vi "RelayControl.vi"(0 "Relay Task":refnum<k21>, 5 "error in":errorcluster, 7 "Battery Select (0: Off)":i32, 9 "NHR VISA":refnum<visa-resource-name>, 11 "NHR error in":errorcluster caption="NHR error in (no error)") -> (6 "error out":errorcluster, 10 "NHR Visa out":refnum<visa-resource-name>, 15 "NHR error out":errorcluster)   [LabVIEW 2020]
uses:
  <vilib>/DAQmx/write.llb/DAQmx Write (Digital 1D Bool NChan 1Samp 1Line).vi
  <vilib>/DAQmx/miscellaneous.llb/DAQmx Fill In Error Info.vi
  <instrlib>/NH Research Regenerative Test Series/NH Research Regenerative Test Series.lvlib
panel:
  out "String":string
  out "error out 3":errorcluster
  out "error out 2":errorcluster
  # "0:off, 1:B1 NHR, 2:B2 NHR, 3:B3 NHR, 4:3P NHR, 5:B1 BK, 6:B2 BK, 7:B3 BK, 8:3P BK"
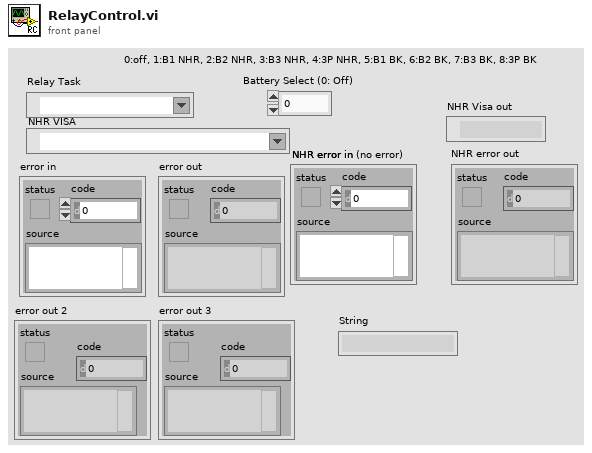
[diagram p1: front panel]
types:
  T1 = cluster{bool, bool, bool, bool, bool, bool, bool}
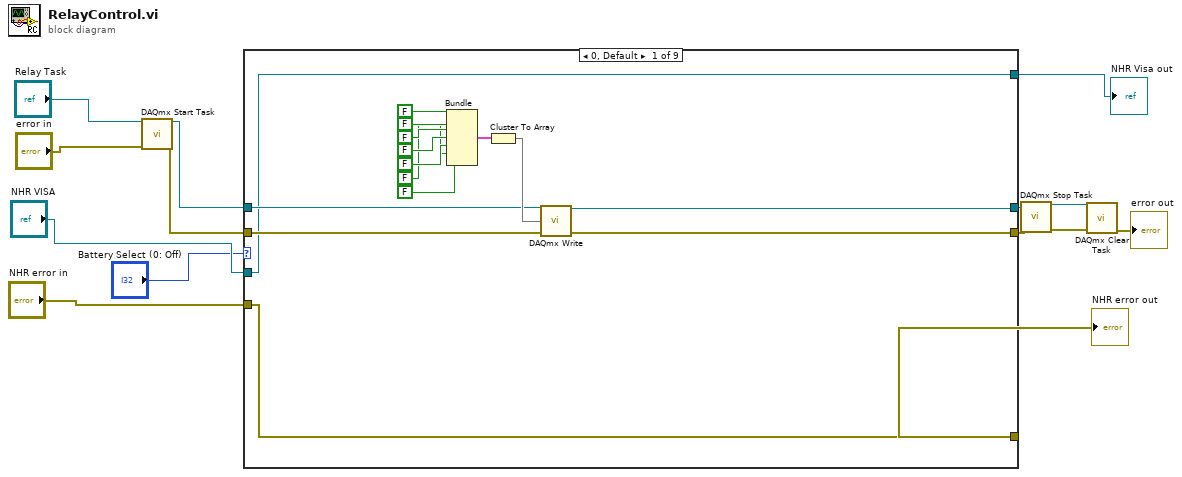
[diagram p0: block diagram]
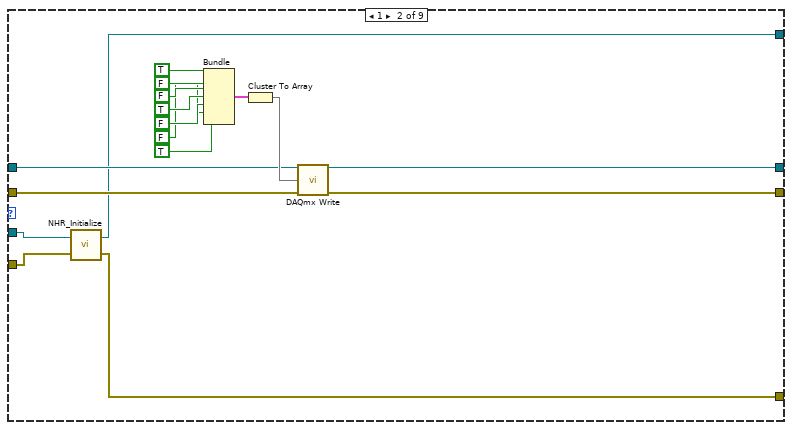
[diagram p2: hidden frame]
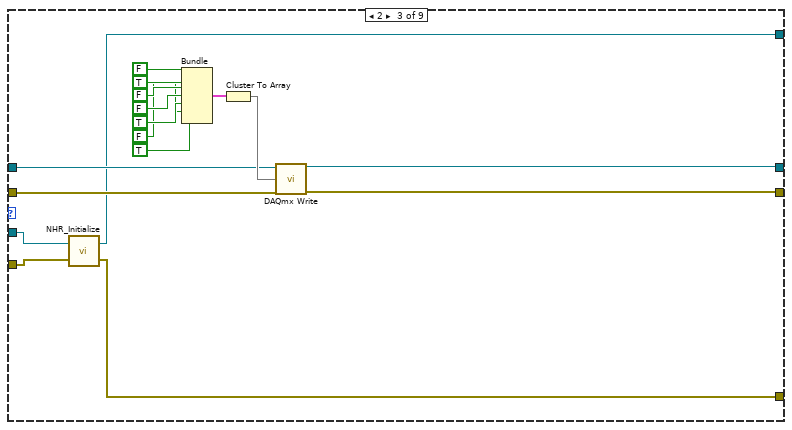
[diagram p3: hidden frame]
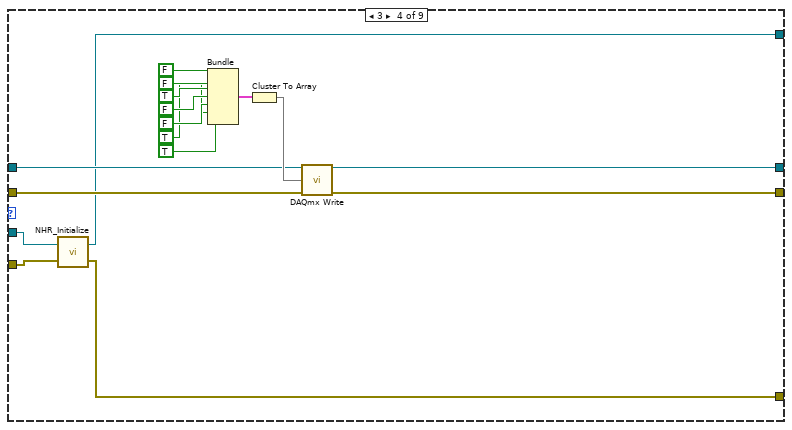
[diagram p4: hidden frame]
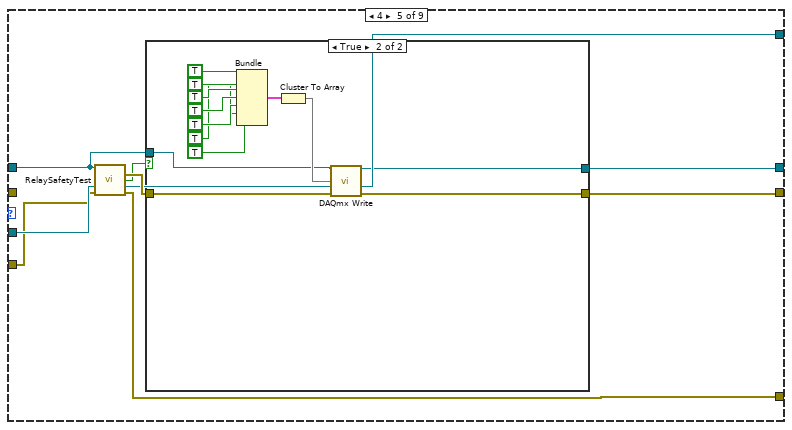
[diagram p5: hidden frame]
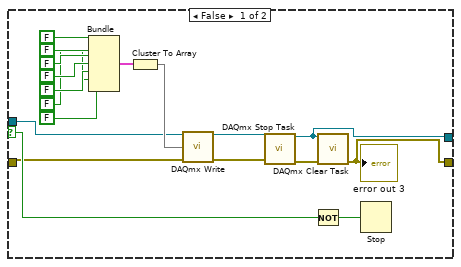
[diagram p6: hidden frame]
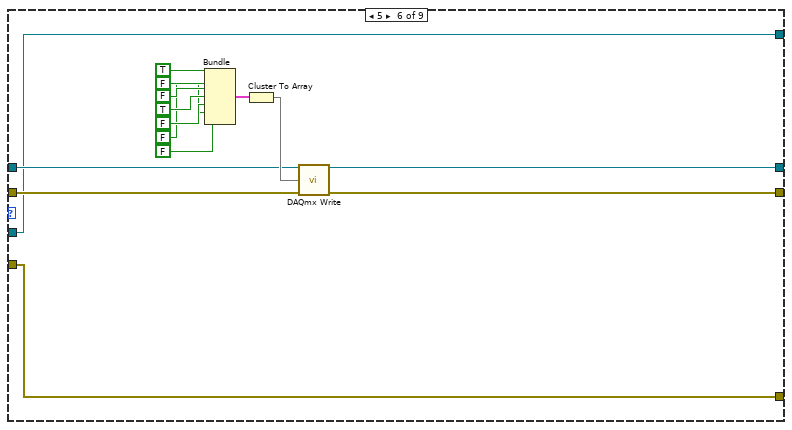
[diagram p7: hidden frame]
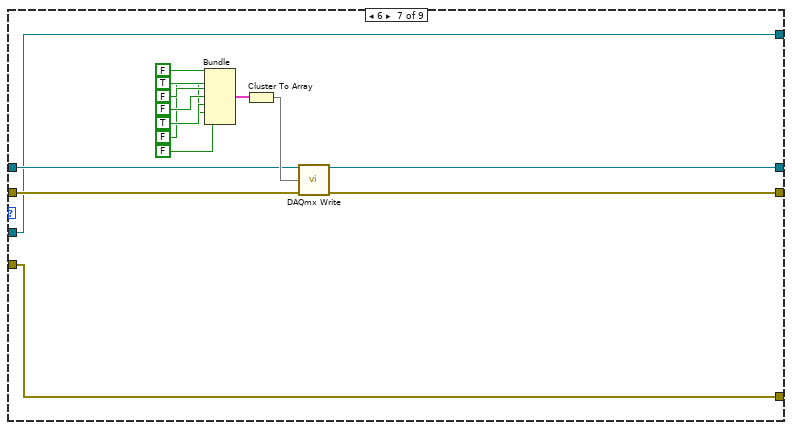
[diagram p8: hidden frame]
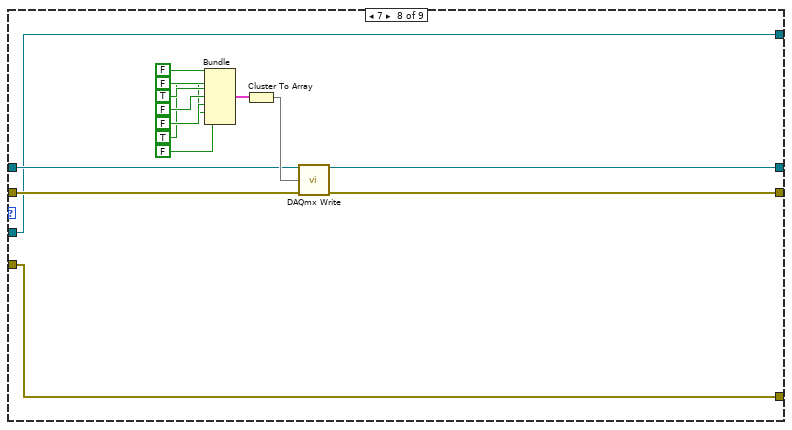
[diagram p9: hidden frame]
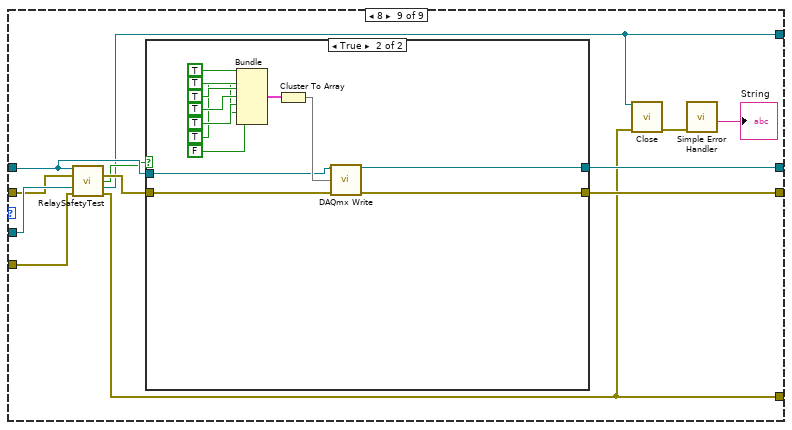
[diagram p10: hidden frame]
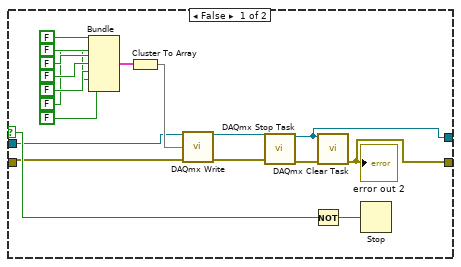
[diagram p11: hidden frame]
diagram:
  n1 = call <vilib>:"DAQmx Start Task.vi"("task/channels in"="Relay Task", "error in"="error in") -> ("task out"=w13:refnum<k21>, "error out"=w12:errorcluster)  [unwired: 12 in]
  n2 = case shown="0, Default" "Battery Select (0: Off)" {
    tunnel: w13 -> [w20 w37 w54 w71 w87 w126 w141 w156 w173]
    tunnel: w12 -> [w19 w36 w53 w70 _ w125 w140 w155 w174]
    tunnel: [w18 w35 w52 w69 w89 w124 w139 w154 w177] -> w8
    tunnel: [w17 w34 w51 w68 w88 w123 w138 w153 w167] -> w7
    tunnel: "NHR VISA" -> [w16 w33 w50 w67 w83 w122 w137 w152 w176]
    tunnel: "NHR error in" -> [w15 w32 w49 w66 w82 w121 w136 w151 w175]
    tunnel: [w16 w31 w48 w65 w85 w122 w137 w152 w168] -> w3
    tunnel: [w15 w30 w47 w64 w84 w121 w136 w151 w166] -> w2
    frame 0, Default {
      n3 = Bundle(FALSE, FALSE, FALSE, FALSE, FALSE, FALSE, FALSE) -> (w29:T1)  [unwired: 1 in]
      n4 = Cluster To Array(cluster=w29) -> (array=w21:bool[])
      n5 = call-poly <vilib>:"DAQmx Write.vi"("task/channels in"=w20, "data"=w21, "error in"=w19) -> ("task out"=w18:refnum<k21>, "error out"=w17:errorcluster)  [unwired: 10 in, 1 out]
    }
    frame 1 {
      n6 = call "NHR_Initialize.vi"("NHR error in"=w32, "NHR VISA"=w33) -> ("NHR error out"=w30:errorcluster, "NHR VISA out"=w31:refnum<visa-resource-name>)
      n7 = Bundle(TRUE, FALSE, FALSE, TRUE, FALSE, FALSE, TRUE) -> (w46:T1)  [unwired: 1 in]
      n8 = Cluster To Array(cluster=w46) -> (array=w38:bool[])
      n9 = call-poly <vilib>:"DAQmx Write.vi"("task/channels in"=w37, "data"=w38, "error in"=w36) -> ("task out"=w35:refnum<k21>, "error out"=w34:errorcluster)  [unwired: 10 in, 1 out]
    }
    frame 2 {
      n10 = call "NHR_Initialize.vi"("NHR error in"=w49, "NHR VISA"=w50) -> ("NHR error out"=w47:errorcluster, "NHR VISA out"=w48:refnum<visa-resource-name>)
      n11 = Bundle(FALSE, TRUE, FALSE, FALSE, TRUE, FALSE, TRUE) -> (w63:T1)  [unwired: 1 in]
      n12 = Cluster To Array(cluster=w63) -> (array=w55:bool[])
      n13 = call-poly <vilib>:"DAQmx Write.vi"("task/channels in"=w54, "data"=w55, "error in"=w53) -> ("task out"=w52:refnum<k21>, "error out"=w51:errorcluster)  [unwired: 10 in, 1 out]
    }
    frame 3 {
      n14 = call "NHR_Initialize.vi"("NHR error in"=w66, "NHR VISA"=w67) -> ("NHR error out"=w64:errorcluster, "NHR VISA out"=w65:refnum<visa-resource-name>)
      n15 = Bundle(FALSE, FALSE, TRUE, FALSE, FALSE, TRUE, TRUE) -> (w80:T1)  [unwired: 1 in]
      n16 = Cluster To Array(cluster=w80) -> (array=w72:bool[])
      n17 = call-poly <vilib>:"DAQmx Write.vi"("task/channels in"=w71, "data"=w72, "error in"=w70) -> ("task out"=w69:refnum<k21>, "error out"=w68:errorcluster)  [unwired: 10 in, 1 out]
    }
    frame 4 {
      n18 = call "RelaySafetyTest.vi"("Relay Task"=w87, "NI VISA"=w83, "NHR error in"=w82) -> ("error out"=w86:errorcluster, "Safe to connect"=w81:bool, "NHR Visa out"=w85:refnum<visa-resource-name>, "NHR error out"=w84:errorcluster)  [unwired: 9 in]
      n19 = case shown="True" w81 {
        selector: w81 -> [w94 _]
        tunnel: [w92 w111] -> w89
        tunnel: [w91 w110] -> w88
        tunnel: w87 -> [w93 w109]
        tunnel: w86 -> [w90 w108]
        frame False {
          n20 = Bundle(FALSE, FALSE, FALSE, FALSE, FALSE, FALSE, FALSE) -> (w105:T1)  [unwired: 1 in]
          n21 = Cluster To Array(cluster=w105) -> (array=w97:bool[])
          n22 = call-poly <vilib>:"DAQmx Write.vi"("task/channels in"=w93, "data"=w97, "error in"=w90) -> ("task out"=w96:refnum<k21>, "error out"=w95:errorcluster)  [unwired: 10 in, 1 out]
          n23 = call <vilib>:"DAQmx Stop Task.vi"("task/channels in"=w96, "error in"=w95) -> ("task out"=w92:refnum<k21>, "error out"=w107:errorcluster)  [unwired: 12 in]
          n24 = Not(x=w94) -> (.not. x?=w106:bool)
          n25 = call <vilib>:"DAQmx Clear Task.vi"("task in"=w92, "error in"=w107) -> ("error out"=w91:errorcluster)  [unwired: 13 in]
          "error out 3" <- w91
          n26 = Stop(stop? (T)=w106) -> ()
        }
        frame True {
          n27 = Bundle(TRUE, TRUE, TRUE, TRUE, TRUE, TRUE, TRUE) -> (w120:T1)  [unwired: 1 in]
          n28 = Cluster To Array(cluster=w120) -> (array=w112:bool[])
          n29 = call-poly <vilib>:"DAQmx Write.vi"("task/channels in"=w109, "data"=w112, "error in"=w108) -> ("task out"=w111:refnum<k21>, "error out"=w110:errorcluster)  [unwired: 10 in, 1 out]
        }
      }
    }
    frame 5 {
      n30 = Bundle(TRUE, FALSE, FALSE, TRUE, FALSE, FALSE, FALSE) -> (w135:T1)  [unwired: 1 in]
      n31 = Cluster To Array(cluster=w135) -> (array=w127:bool[])
      n32 = call-poly <vilib>:"DAQmx Write.vi"("task/channels in"=w126, "data"=w127, "error in"=w125) -> ("task out"=w124:refnum<k21>, "error out"=w123:errorcluster)  [unwired: 10 in, 1 out]
    }
    frame 6 {
      n33 = Bundle(FALSE, TRUE, FALSE, FALSE, TRUE, FALSE, FALSE) -> (w150:T1)  [unwired: 1 in]
      n34 = Cluster To Array(cluster=w150) -> (array=w142:bool[])
      n35 = call-poly <vilib>:"DAQmx Write.vi"("task/channels in"=w141, "data"=w142, "error in"=w140) -> ("task out"=w139:refnum<k21>, "error out"=w138:errorcluster)  [unwired: 10 in, 1 out]
    }
    frame 7 {
      n36 = Bundle(FALSE, FALSE, TRUE, FALSE, FALSE, TRUE, FALSE) -> (w165:T1)  [unwired: 1 in]
      n37 = Cluster To Array(cluster=w165) -> (array=w157:bool[])
      n38 = call-poly <vilib>:"DAQmx Write.vi"("task/channels in"=w156, "data"=w157, "error in"=w155) -> ("task out"=w154:refnum<k21>, "error out"=w153:errorcluster)  [unwired: 10 in, 1 out]
    }
    frame 8 {
      n39 = call "RelaySafetyTest.vi"("Relay Task"=w173, "task error in"=w174, "NI VISA"=w176, "NHR error in"=w175) -> ("error out"=w172:errorcluster, "Safe to connect"=w171:bool, "NHR Visa out"=w168:refnum<visa-resource-name>, "NHR error out"=w166:errorcluster)  [unwired: 8 in]
      n40 = case shown="True" w171 {
        selector: w171 -> [w182 _]
        tunnel: [w181 w199] -> w177
        tunnel: [w180 w198] -> w167
        tunnel: w173 -> [w179 w197]
        tunnel: w172 -> [w178 w196]
        frame False {
          n41 = Bundle(FALSE, FALSE, FALSE, FALSE, FALSE, FALSE, FALSE) -> (w193:T1)  [unwired: 1 in]
          n42 = Cluster To Array(cluster=w193) -> (array=w185:bool[])
          n43 = call-poly <vilib>:"DAQmx Write.vi"("task/channels in"=w179, "data"=w185, "error in"=w178) -> ("task out"=w184:refnum<k21>, "error out"=w183:errorcluster)  [unwired: 10 in, 1 out]
          n44 = call <vilib>:"DAQmx Stop Task.vi"("task/channels in"=w184, "error in"=w183) -> ("task out"=w181:refnum<k21>, "error out"=w195:errorcluster)  [unwired: 12 in]
          n45 = Not(x=w182) -> (.not. x?=w194:bool)
          n46 = call <vilib>:"DAQmx Clear Task.vi"("task in"=w181, "error in"=w195) -> ("error out"=w180:errorcluster)  [unwired: 13 in]
          "error out 2" <- w180
          n47 = Stop(stop? (T)=w194) -> ()
        }
        frame True {
          n48 = Bundle(TRUE, TRUE, TRUE, TRUE, TRUE, TRUE, FALSE) -> (w208:T1)  [unwired: 1 in]
          n49 = Cluster To Array(cluster=w208) -> (array=w200:bool[])
          n50 = call-poly <vilib>:"DAQmx Write.vi"("task/channels in"=w197, "data"=w200, "error in"=w196) -> ("task out"=w199:refnum<k21>, "error out"=w198:errorcluster)  [unwired: 10 in, 1 out]
        }
      }
      n51 = call <instrlib>:"Close.vi"("VISA resource name"=w168, "error in (no error)"=w166) -> ("error out"=w169:errorcluster)  [unwired: 13 in]
      n52 = call <vilib>:"Simple Error Handler.vi"("error in (no error)"=w169) -> ("source out"=→"String":string)  [unwired: 4 in, 4 out]
    }
  }
  "NHR Visa out" <- w3
  "NHR error out" <- w2
  n53 = call <vilib>:"DAQmx Stop Task.vi"("task/channels in"=w8, "error in"=w7) -> ("task out"=w11:refnum<k21>, "error out"=w10:errorcluster)  [unwired: 12 in]
  n54 = call <vilib>:"DAQmx Clear Task.vi"("task in"=w11, "error in"=w10) -> ("error out"=→"error out":errorcluster)  [unwired: 13 in]
